vi "test http origin.vi"(8 "error in (no error)":errorcluster) -> (0 "error out":errorcluster, 3 "body":string)   [LabVIEW 2020, in "MCP Server tests.lvlib"]
doc: "A request with a foreign Origin header must be rejected with 403 and a JSON-RPC error with code -32600. A request with a local Origin must be handled normally."
uses:
  MCP Server tests.lvlib
  <vilib>/JDP Science/JSONtext/Next JSON Value.vi
  <vilib>/JDP Science/JSONtext/String Subset.vi
  <vilib>/JDP Science/JSONtext/Parsing/Advance past next JSON Value (inlined COPY).vi
  <vilib>/JDP Science/JSONtext/Parsing/Advance past whitespace.vi
  <vilib>/JDP Science/JSONtext/Parsing/Advance past String.vi
  <vilib>/JDP Science/JSONtext/Parsing/Advance past Number.vi
  <vilib>/JDP Science/JSONtext/Parsing/Advance past Line Ending.vi
  <vilib>/JDP Science/JSONtext/Parsing/Parse Full Path or Item Name.vi
  <vilib>/JDP Science/JSONtext/Parsing/Advance past Array.vi
  <vilib>/JDP Science/JSONtext/Parsing/Advance past Object.vi
  <vilib>/JDP Science/JSONtext/support/Error Cluster From Code.vi
  <vilib>/JDP Science/JSONtext/Offset/Find Item Locations by Path.vi
  <vilib>/addons/_JKI Toolkits/Caraya/classes/Test/Test.lvclass
  <vilib>/addons/_JKI Toolkits/Caraya/classes/Assert/Assert.lvclass
  <vilib>/JDP Science/JSONtext/JSONtext.lvlib
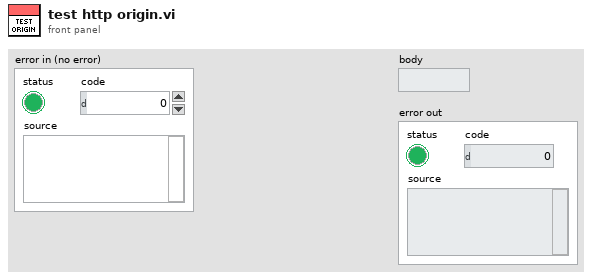
[diagram p1: front panel]
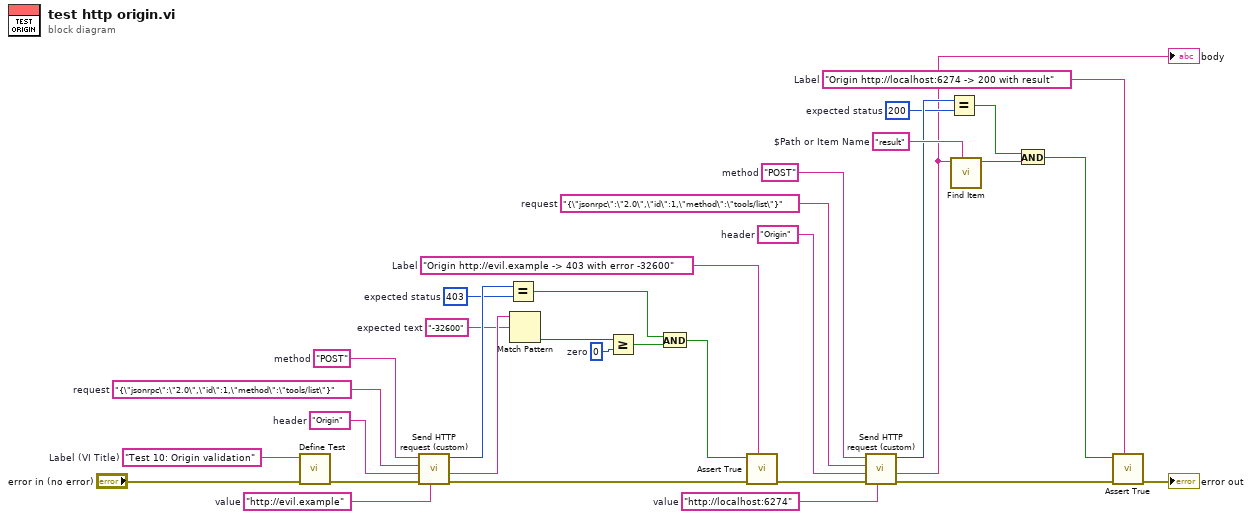
[diagram p0: block diagram]
diagram:
  w3 = "Origin http://localhost:6274 -> 200 with result"  # Label
  w8 = 200  # expected status
  w10 = "result"  # $Path or Item Name
  w12 = "http://localhost:6274"  # value
  w13 = "Origin"  # header
  w14 = "{\"jsonrpc\":\"2.0\",\"id\":1,\"method\":\"tools/list\"}"  # request
  w15 = "POST"  # method
  w16 = "Origin http://evil.example -> 403 with error -32600"  # Label
  w21 = 0  # zero
  w23 = "-32600"  # expected text
  w25 = 403  # expected status
  w28 = "http://evil.example"  # value
  w29 = "Origin"  # header
  w30 = "{\"jsonrpc\":\"2.0\",\"id\":1,\"method\":\"tools/list\"}"  # request
  w31 = "POST"  # method
  w33 = "Test 10: Origin validation"  # Label (VI Title)
  n1 = call <vilib>:"Define Test.vi"("error in (no error)"="error in (no error)", "Label (VI Title)"=w33) -> ("error out"=w27:errorcluster)  [unwired: 8 in, 1 out]
  n2 = call "Send HTTP request (custom).vi"("value"=w28, "error in (no error)"=w27, "header"=w29, "request"=w30, "method"=w31) -> ("error out"=w17:errorcluster, "response"=w24:string, "status code"=w26:i32)  [unwired: 3 in, 1 out]
  n3 = Equal?(x=w26, y=w25) -> (x = y?=w20:bool)
  n4 = Match Pattern(string=w24, regular expression=w23) -> (offset past match=w22:i32)  [unwired: 1 in, 3 out]
  n5 = Greater Or Equal?(x=w22, y=w21) -> (x >= y?=w19:bool)
  n6 = And(x=w20, y=w19) -> (x .and. y?=w18:bool)
  n7 = call <vilib>:"Assert True.vi"("Label"=w16, "error in (no error)"=w17, "True?"=w18) -> ("error out"=w11:errorcluster)  [unwired: 7 in, 1 out]
  n8 = call "Send HTTP request (custom).vi"("value"=w12, "error in (no error)"=w11, "header"=w13, "request"=w14, "method"=w15) -> ("error out"=w4:errorcluster, "response"=w2:string, "status code"=w9:i32)  [unwired: 3 in, 1 out]
  "body" <- w2
  n9 = Equal?(x=w9, y=w8) -> (x = y?=w7:bool)
  n10 = call <vilib>:"Find Item.vi"("$Path or Item Name"=w10, "JSON"=w2) -> ("Found"=w6:bool)  [unwired: 6 in, 3 out]
  n11 = And(x=w7, y=w6) -> (x .and. y?=w5:bool)
  n12 = call <vilib>:"Assert True.vi"("Label"=w3, "error in (no error)"=w4, "True?"=w5) -> ("error out"=→"error out":errorcluster)  [unwired: 7 in, 1 out]
